vi "set endianness.vi"(8 "error in":errorcluster, 10 "byte orders":T4[](array[typedef]), 11 "config in":T1[](array[typedef])) -> (0 "error out":errorcluster, 3 "config out":T1[](array[typedef]))   [LabVIEW 2013, in "Profibus Module runtime.lvclass"]
uses:
  Profibus Module runtime.lvclass
  configuration/endianness setting.ctl
  profibus slave configuration.ctl
  profibus mapping configuration.ctl
  <vilib>/NI/Tag Bus/tag/Data Type.ctl
  configuration/Profibus Module configuration.lvclass
  <vilib>/NI/Tag Bus/tag/tag descriptor.lvclass
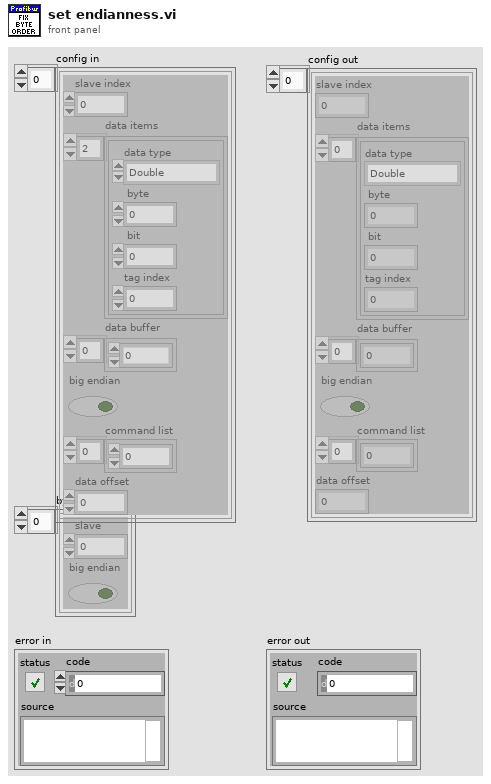
[diagram p1: front panel]
types:
  T1 = typedef "Profibus Module runtime.lvclass/profibus slave configuration.ctl" = cluster{"slave index":i8, "data items":T2[], "data buffer":u8[], "big endian":bool, "command list":u32[], "data offset":u8}
  T2 = typedef "Profibus Module runtime.lvclass/profibus mapping configuration.ctl" = cluster{"data type":T3, " byte":i32, " bit":i32, "tag index":i32}
  T3 = typedef "tag bus.lvlib/tag descriptor.lvclass/Data Type.ctl" = enum16{"Double", "Single", "I64", "I32", "I16", "I8", "U64", "U32", "U16", "U8", "Boolean", "String", "Array of Double", "Array of Single", "Array of I64", "Array of I32", "Array of I16", "Array of I8", "Array of U64", "Array of U32", "Array of U16", "Array of U8", "Array of Boolean", "Array of String"}
  T4 = typedef "Profibus Module configuration.lvclass/endianness setting.ctl" = cluster{"slave":i8, "big endian":bool}
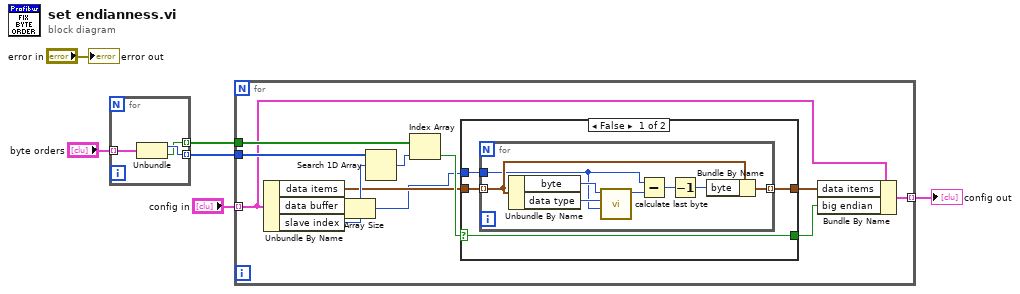
[diagram p0: block diagram]
diagram:
  n1 = for {
    tunnel: "byte orders" -> [w9] mode=indexing
    tunnel: [w8] -> w4 mode=indexing
    tunnel: [w7] -> w3 mode=indexing
    n2 = Unbundle(w9) -> ("slave"=w8:i8, "big endian"=w7:bool)
  }
  n3 = for {
    tunnel: "config in" -> [w17] mode=indexing
    tunnel: w4 -> [w21]
    tunnel: w3 -> [w19]
    tunnel: [w16] -> w2 mode=indexing
    n4 = Unbundle By Name(w17) -> ("data items"=w12:T2[], "data buffer"=w11:u8[], "slave index"=w20:i8)
    n5 = Array Size(array=w11) -> (size(s)=w10:i32)
    n6 = Search 1D Array(1D array=w21, element=w20) -> (index of element=w18:i32)  [unwired: 1 in]
    n7 = Index Array(array=w19, index=w18) -> (element=w15:bool)
    n8 = case shown="False" w15 {
      selector: w15 -> [w25 w35]
      tunnel: [w25 w35] -> w14
      tunnel: [w22 w34] -> w13
      tunnel: w12 -> [w24 w34]
      tunnel: w10 -> [w23 _]
      frame False {
        n9 = for {
          tunnel: w24 -> [w31] mode=indexing
          tunnel: w23 -> [w26]
          tunnel: [w30] -> w22 mode=indexing
          n10 = Unbundle By Name(w31) -> ("byte"=w33:i32, "data type"=w32:T3)
          n11 = call "calculate last byte.vi"("buffer length"=w26, "type"=w32, "byte in"=w33) -> ("last byte"=w29:i32)  [unwired: 8 in]
          n12 = Subtract(x=w26, y=w29) -> (x-y=w28:i32)
          n13 = Decrement(x=w28) -> (x-1=w27:i32)
          n14 = Bundle By Name(cluster=w31, "byte"=w27) -> (w30:T2)
        }
      }
      frame True {
      }
    }
    n15 = Bundle By Name(cluster=w17, "data items"=w13, "big endian"=w14) -> (w16:T1)
  }
  "config out" <- w2
  "error out" <- "error in"
